vi "SPARK Set Sensor Position.vi"(7 "Sensor (Primary Encoder)":enum16{"Primary Encoder", "Alt/Ext Encoder"}(ring), 8 "error in":errorcluster, 10 "Position":dbl, 11 "Spark refnum":T1) -> (0 "error out":errorcluster, 3 "Spark refnum":T1)   [LabVIEW 2023, in "REVLibDriver.lvlib"]
doc: "Set the position of a sensor. By default the units are 'rotations' and can be changed by a scale factor setting the sensor's position conversion factor."
uses:
  <vilib>/REVLibDriver/REVLibDriver.lvlib
  <vilib>/REV Custom Controls/REVSparkRefnum.ctl
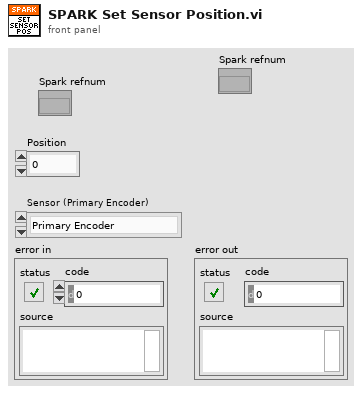
[diagram p1: front panel]
types:
  T1 = typedef "REVLibDriver.lvlib/REVSparkRefnum.ctl" = refnum<k20>
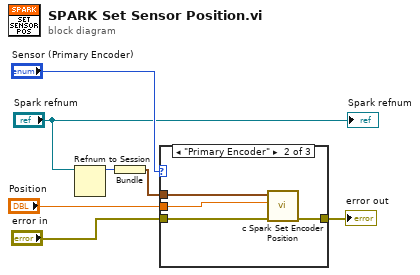
[diagram p0: block diagram]
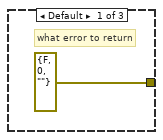
[diagram p2: hidden frame]
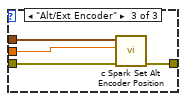
[diagram p3: hidden frame]
diagram:
  n1 = Refnum to Session(7:"Spark refnum") -> (3:w2:u64)  [unwired: 1 in, 1 out]
  n2 = Bundle("Session"=w2) -> (w1:cluster{"Session":u64})  [unwired: 1 in]
  n3 = case shown="\"Primary Encoder\"" "Sensor (Primary Encoder)" {
    tunnel: "Position" -> [_ w12 w16]
    tunnel: "error in" -> [_ w11 w14]
    tunnel: [errorcluster {"status"=FALSE, "code"=0, "source"=""} ("error out") w10 w15] -> w4
    tunnel: w1 -> [_ w9 w13]
    frame Default {
      # "what error to return"
    }
    frame "Primary Encoder" {
      n4 = call <vilib>:"c Spark Set Encoder Position.vi"("error in (no error)"=w11, "position"=w12, "handle"=w9) -> ("error out"=w10:errorcluster)  [unwired: 6 in, 2 out]
    }
    frame "Alt/Ext Encoder" {
      n5 = call <vilib>:"c Spark Set Alt Encoder Position.vi"("error in (no error)"=w14, "position"=w16, "handle"=w13) -> ("error out"=w15:errorcluster)  [unwired: 6 in, 2 out]
    }
  }
  "error out" <- w4
  "Spark refnum" <- "Spark refnum"
